vi "连续采集 - L1.vi"() -> ()   [LabVIEW 2017]
doc: "该范例演示了如何使用DAQmx设备进行连续带缓冲的电压测量。\n\n关于如何连接信号至DAQ设备，请查阅设备手册。"
uses:
  <vilib>/DAQmx/read.llb/DAQmx Read (Analog 2D DBL NChan NSamp).vi
  <vilib>/Analysis/baseanly.llb/Mean (DBL).vi
  <vilib>/DAQmx/write.llb/DAQmx Write (Digital U32 1Chan 1Samp).vi
  <vilib>/DAQmx/create/channels.llb/DAQmx Create Channel (DO-Digital Output).vi
  <vilib>/DAQmx/create/channels.llb/DAQmx Create Channel (AI-Voltage-Basic).vi
  <vilib>/DAQmx/configure/timing.llb/DAQmx Timing (Sample Clock).vi
  <vilib>/DAQmx/miscellaneous.llb/DAQmx Fill In Error Info.vi
  <resource>/objmgr/daqmx.rc
  <vilib>/Analysis/NI_AALBase.lvlib
  <vilib>/ptbypt/NI_PtbyPt.lvlib
panel:
  out "当前时间":timestamp
  out "实际间隔(s)":dbl=0.08 format="%.2g"
  out "显示队列中元素数量":i32
  in  "温度保存间隔(s)":dbl=0.08 format="%.2g"
  in  "校准间隔(s)":dbl=325.0
  out "mean":dbl caption="均值" format="%.7f"
  out "min value":dbl caption="最小值" format="%.7f"
  out "x-y":dbl
  out "校准进度":dbl(slide) scale=0.0..1.0 scale format="%%%#_6g"
  in  "信号采集设备":tag="Dev1"
  in  "波形查看":T1(tab)
  out "单环33":dbl
  out "单环22":dbl
  out "单环2":dbl[](graph)
  out "单环11":dbl
  out "单环3":dbl[](graph)
  out "单环1":dbl[](graph)
  out "单环55":dbl
  out "单环44":dbl
  out "单环5":dbl[](graph)
  out "单环4":dbl[](graph)
  out "N35":dbl=nan
  out "N34":dbl=nan
  out "N45":dbl=nan
  out "差分35":dbl[](graph)
  out "差分34":dbl[](graph)
  out "差分45":dbl[](graph)
  out "N25":dbl=nan
  out "N24":dbl=nan
  out "N23":dbl=nan
  out "差分25":dbl[](graph)
  out "差分24":dbl[](graph)
  out "差分23":dbl[](graph)
  out "N14":dbl=nan
  out "N13":dbl=nan
  out "N12":dbl=nan
  out "差分14":dbl[](graph)
  out "差分13":dbl[](graph)
  out "差分12":dbl[](graph)
  out "校准值":dbl[](array[numeric])
  out "N15":dbl=nan
  out "差分15":dbl[](graph)
  in  "开始":bool
  in  "波长":i32(ring)=3 items=["0"=-1, "1050"=0, "1213"=1, "1314"=2, "1409"=3, "1550"=4, "1609"=5]
  out "Order queue Name":string
  out "Inter queue Name":string
  out "系统标题":string
  out "序号":string
  in  "停止":bool
  # "RTC---"
  # "单环1"
  # "单环2"
  # "单环3"
  # "单环4"
  # "单环5"
  # "差分45"
  # "差分34"
  # "差分35"
  # "差分23"
  # "差分24"
  # "差分25"
  # "差分12"
  # "差分13"
  # "差分14"
  # "差分15"
  # "1环"
  # "2环"
  # "3环"
  # "4环"
  # "5环"
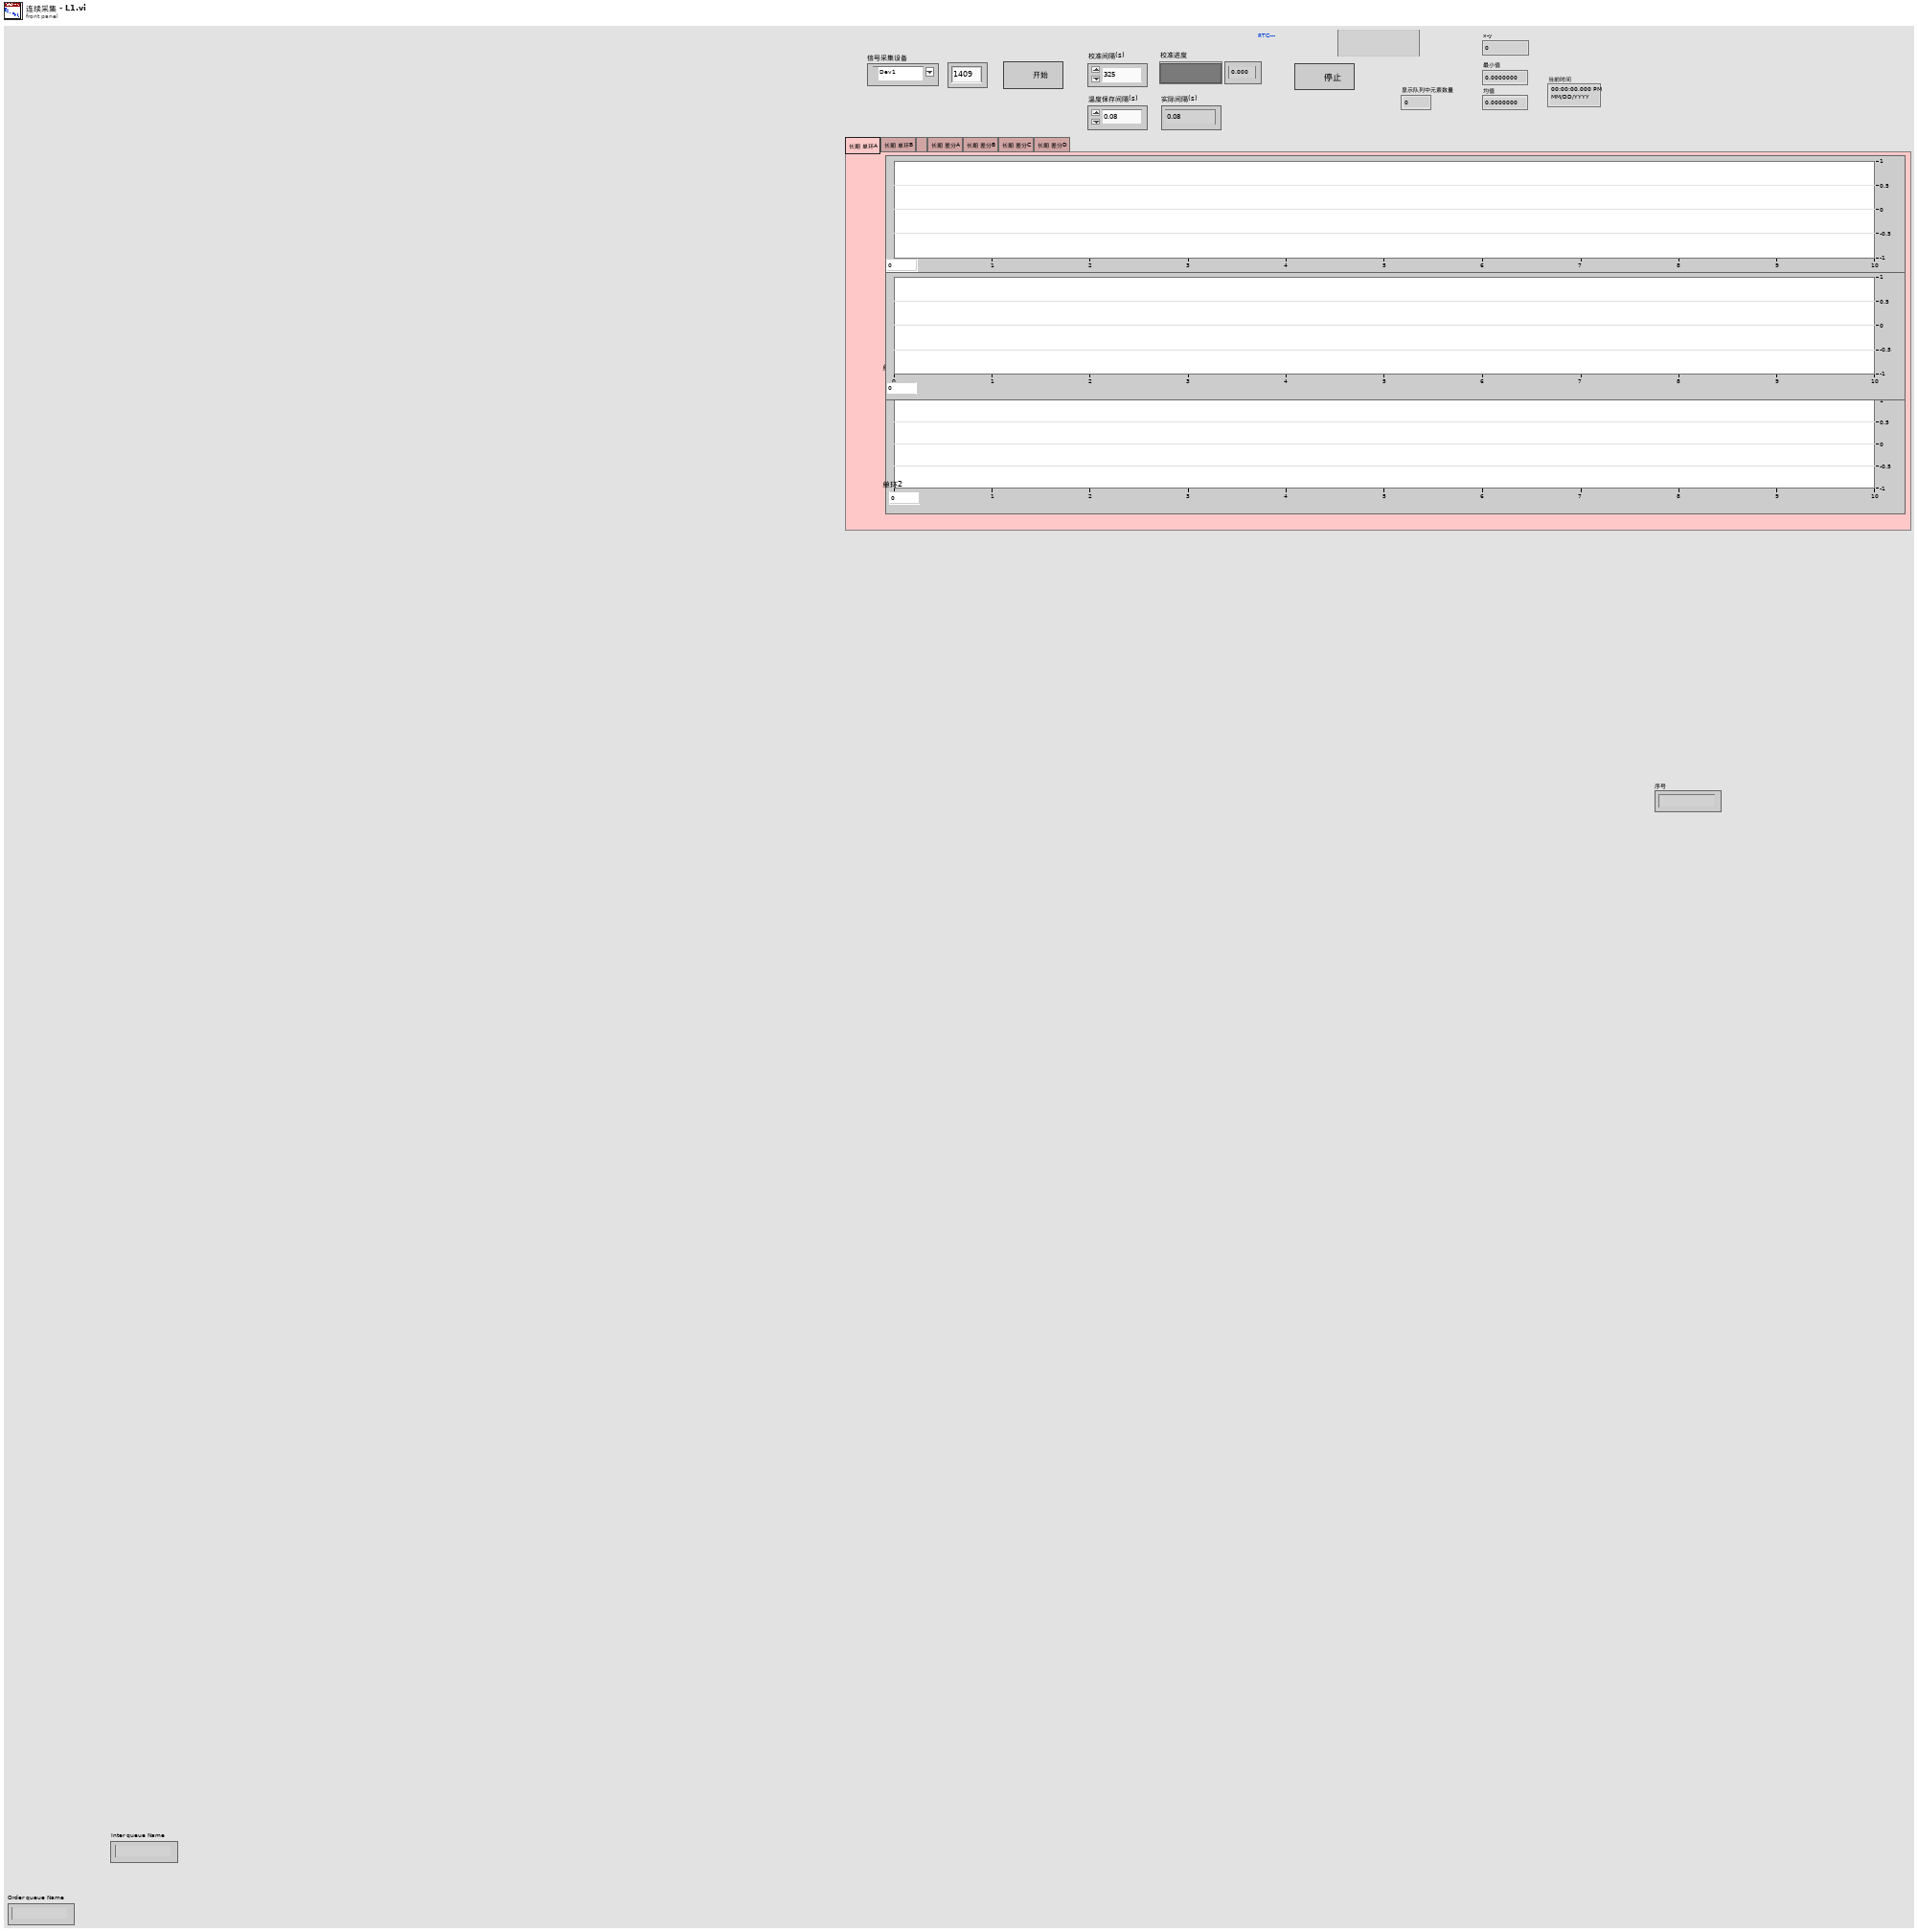
[diagram p1: front panel]
types:
  T1 = enum32{"长期 单环A", "长期 单环B", "  ", "长期 差分A", "长期 差分B", "长期 差分C", "长期 差分D"}
  T2 = cluster{"校准时间":timestamp, "tdms index":refnum<k34>, "Temp Title":string[], "温度保存间隔":dbl}
  T3 = typedef "用户事件自定义控件.ctl" = cluster{"消息":string, "指示":bool, "数据":dbl}
  T4 = cluster{"输入任务":refnum<k21>, "采样数":i32, "数字任务":refnum<k21>, "校准时间":timestamp, "校准值":dbl[], "数据路径":path}
  T5 = enum16{"open", "open or create", "create or replace", "create", "open (read-only)"}
  T6 = cluster{"温度采集":dbl[], "温度控制":dbl[], "压力测量":dbl[], "步进电机":dbl[], "湿度测量":dbl[], "LD温控":dbl[]}
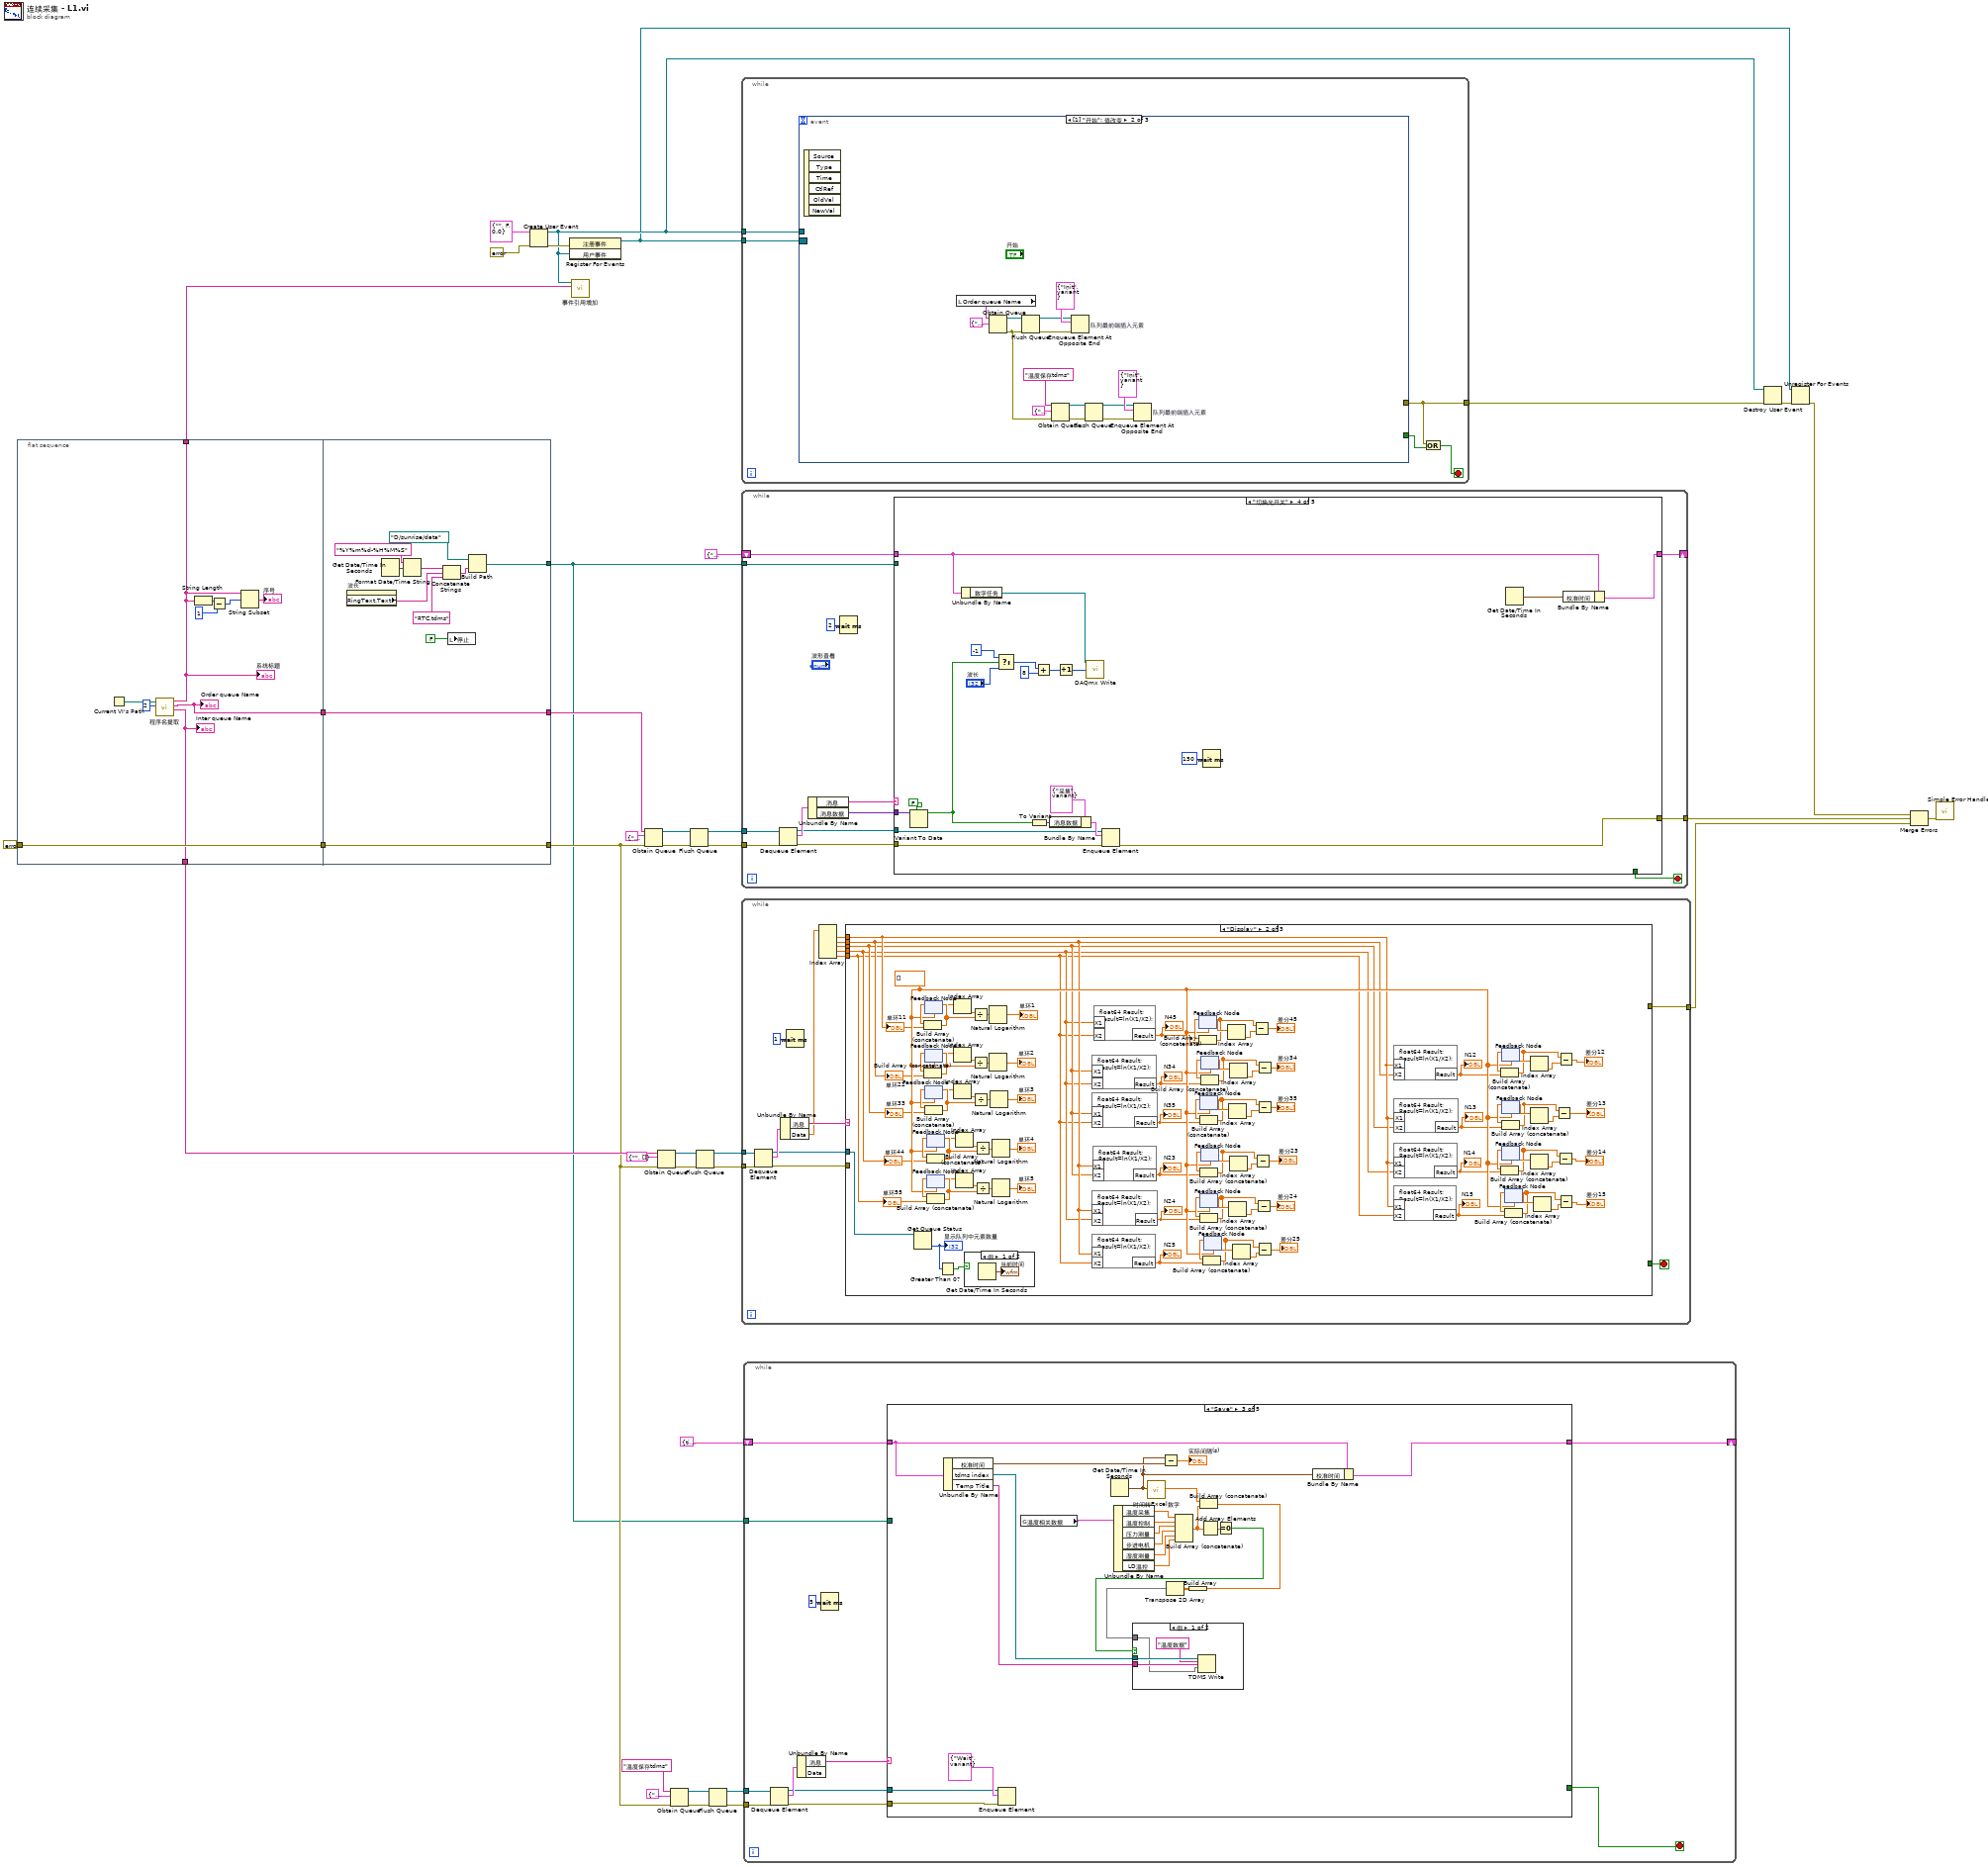
[diagram p0: block diagram]
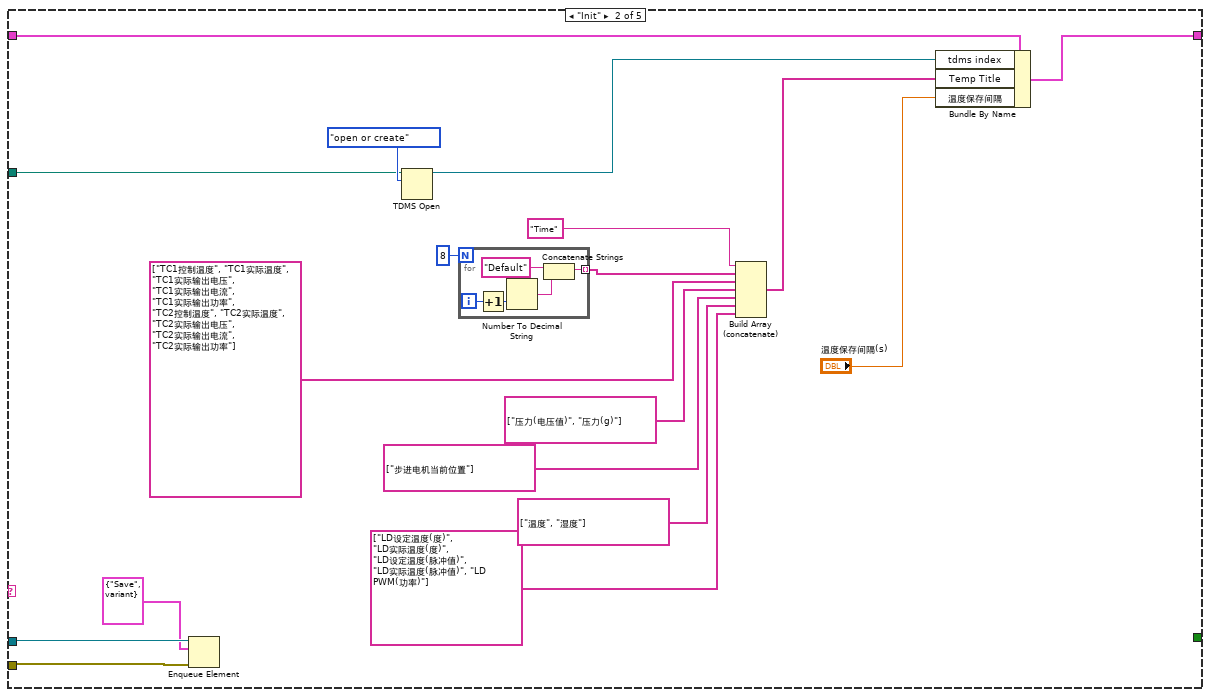
[diagram p3: hidden frame]
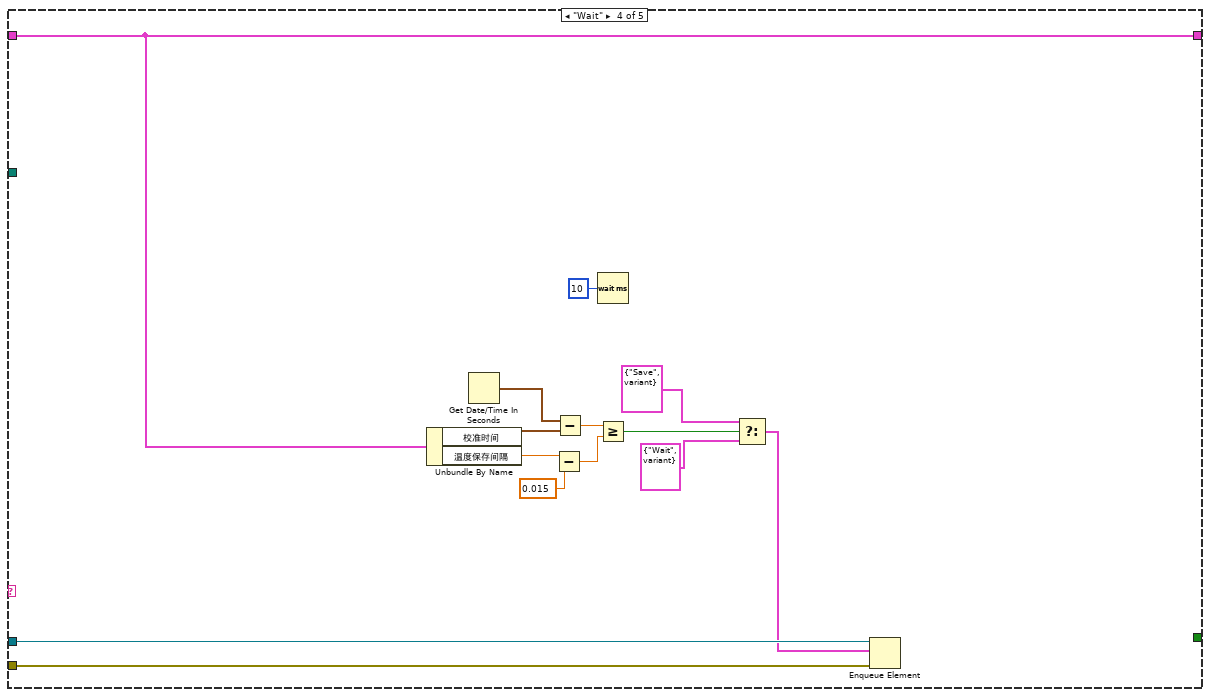
[diagram p5: hidden frame]
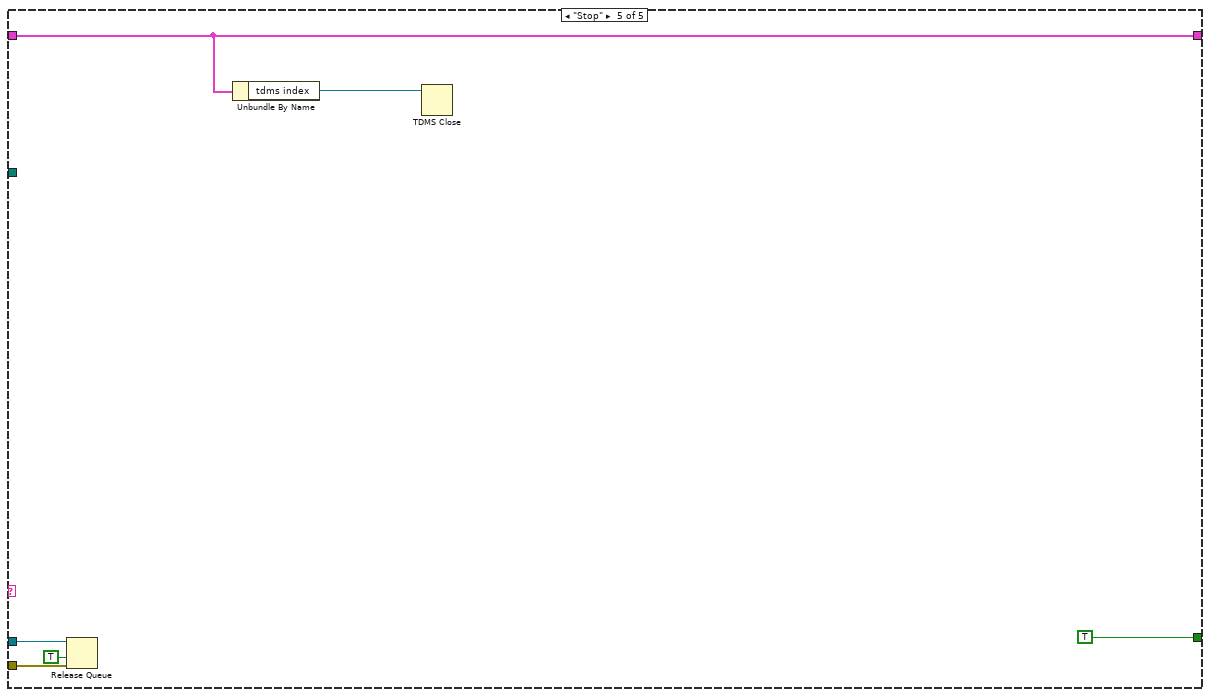
[diagram p6: hidden frame]
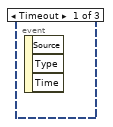
[diagram p7: hidden frame]
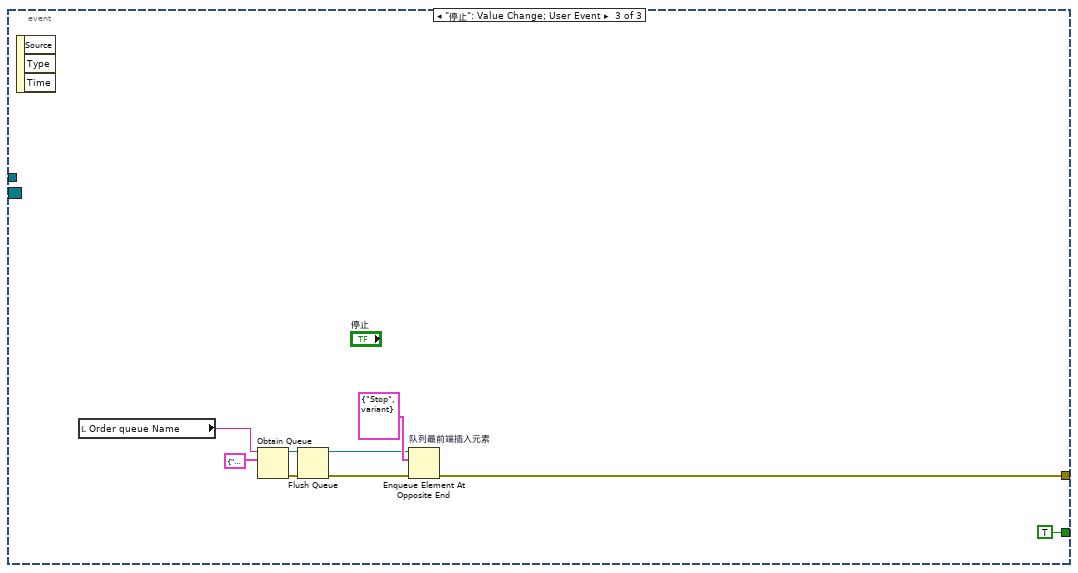
[diagram p8: hidden frame]
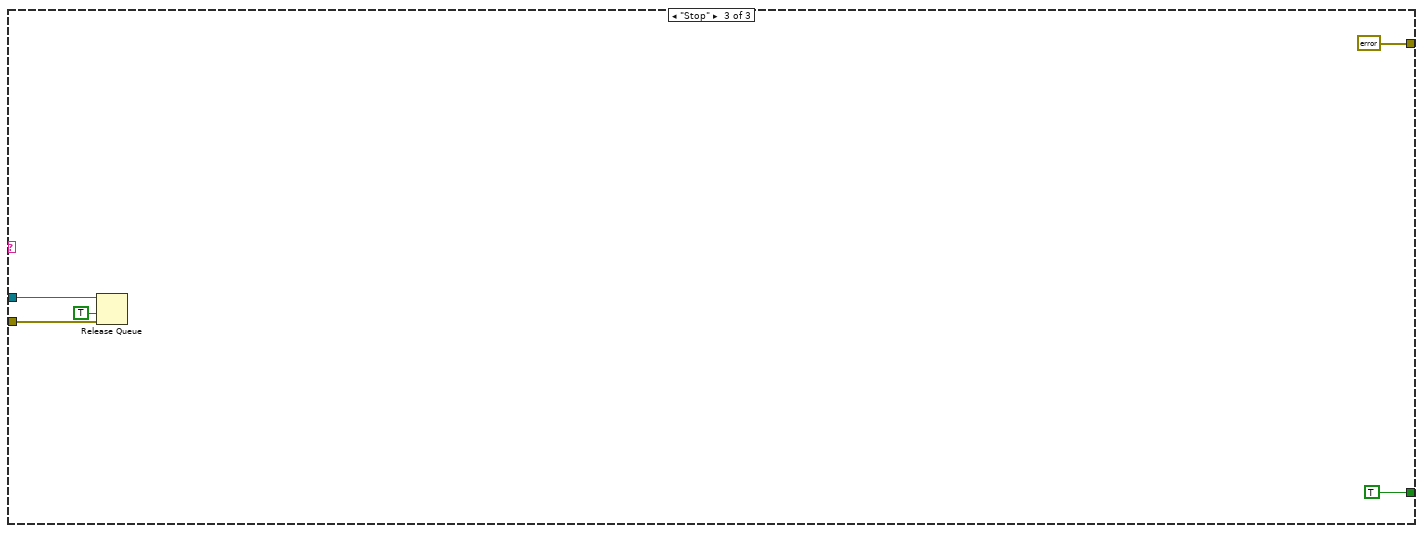
[diagram p11: hidden frame]
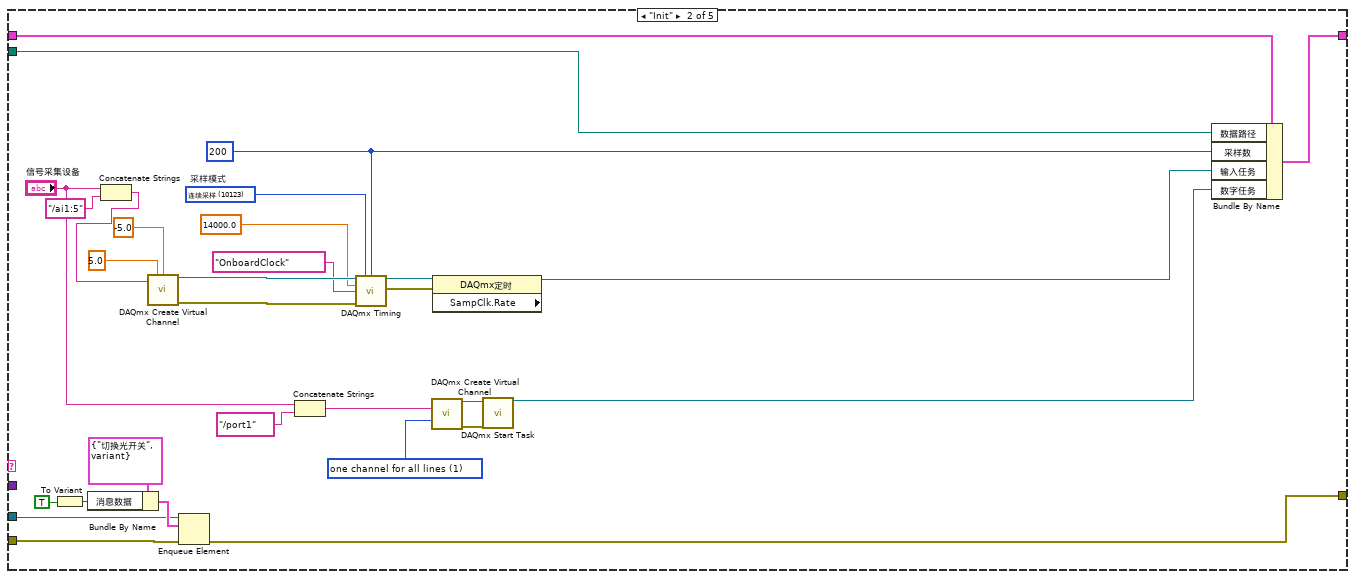
[diagram p13: hidden frame]
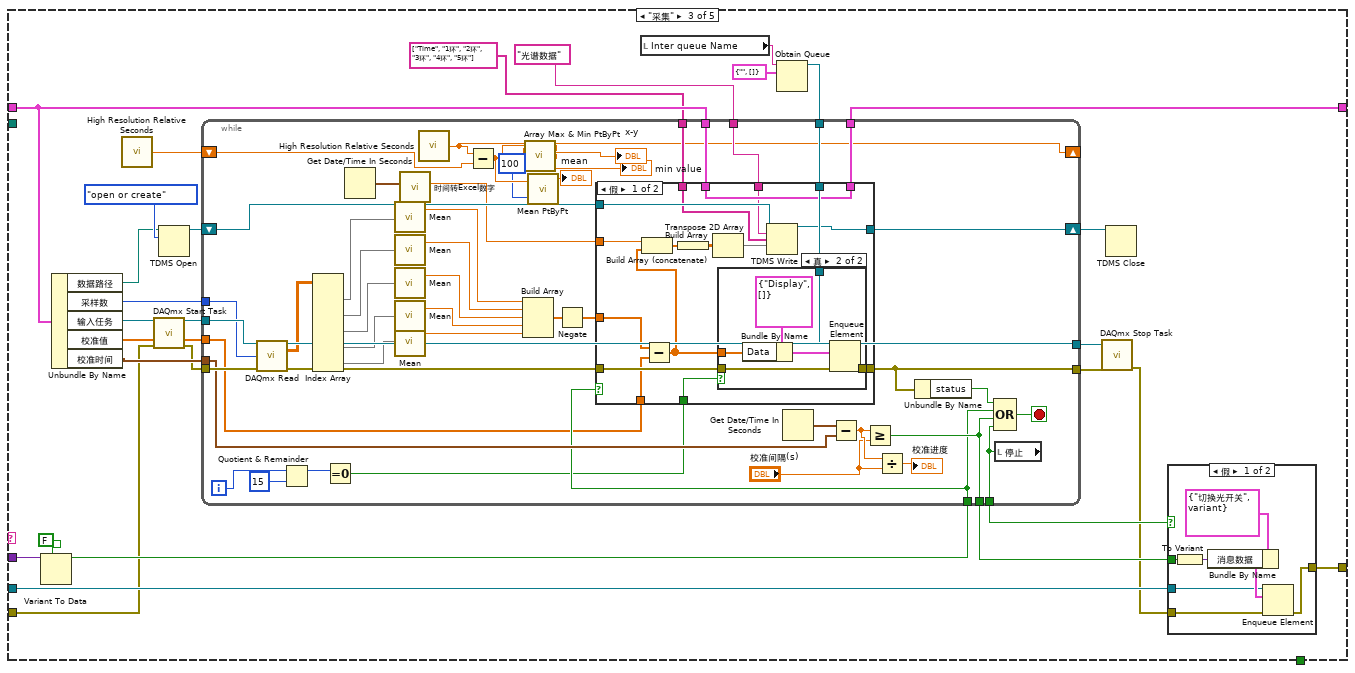
[diagram p14: hidden frame]
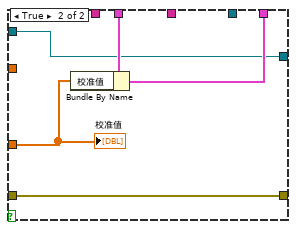
[diagram p17: hidden frame]
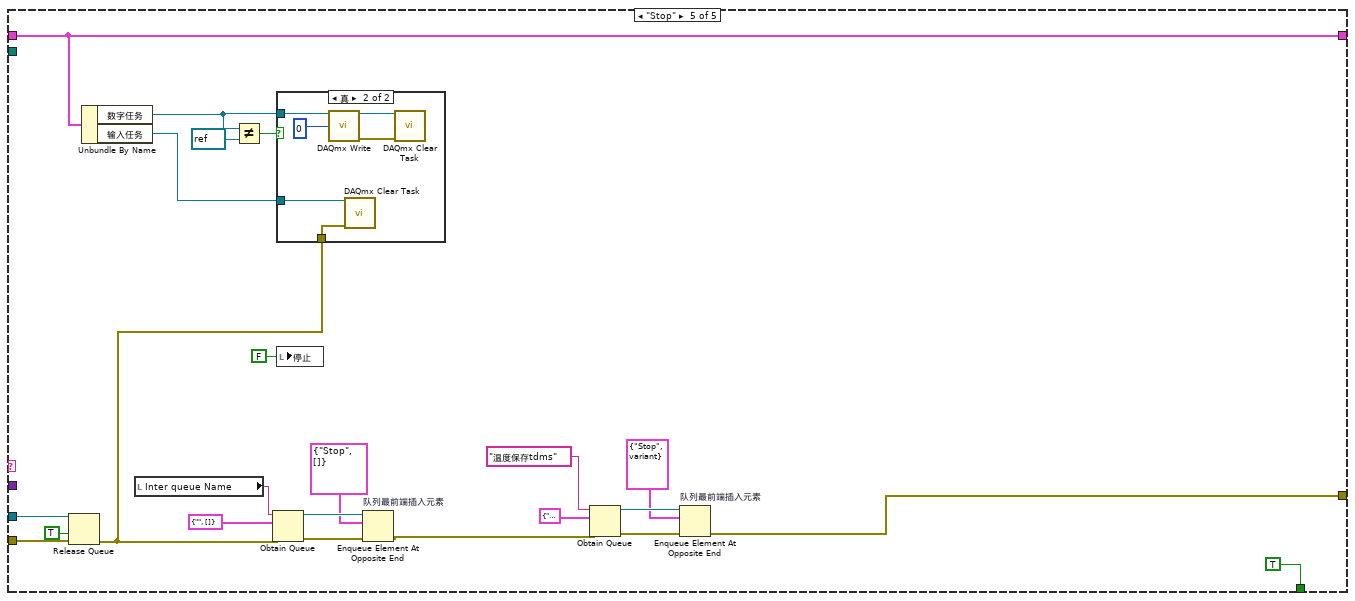
[diagram p18: hidden frame]
diagram:
  n1 = flat-sequence {
    tunnel: errorcluster {"status"=FALSE, "code"=0, "source"=""} ("错误常量") -> [w47]
    tunnel: [w47] -> w37
    tunnel: [w40] -> w24
    tunnel: [w39] -> w36
    tunnel: [w38] -> w16
    tunnel: [w58] -> w3
    tunnel: w37 -> [w58]
    tunnel: [w57] -> w31
    tunnel: w36 -> [w57]
    tunnel: [w50] -> w1
    frame #0 {
      n2 = Current VI's Path() -> (path=w46:path)
      n3 = call "程序名提取.vi"("标识长度"=2 ("长度"), "当前程序路径"=w46) -> ("Inter queue"=w38:string, "Order queue"=w39:string, "系统标题"=w40:string)  [unwired: 7 in]
      "Order queue Name" <- w39
      "Inter queue Name" <- w38
      "系统标题" <- w40
      n4 = String Length(string=w40) -> (length=w43:i32)
      n5 = Subtract(x=w43, y=1) -> (x-y=w44:i32)
      n6 = String Subset(string=w40, offset (0)=w44) -> (substring=→"序号":string)  [unwired: 1 in]
    }
    frame #1 {
      n7 = property on="波长" class="Ring (严格)"() -> ("RingText.Text"=w48:string)  [unwired: 2 in, 2 out]
      n8 = Get Date/Time In Seconds() -> (seconds since 1Jan1904=w52:timestamp)
      n9 = Format Date/Time String(time format string (%c)="%Y%m%d-%H%M%S" ("时间格式字符串(%c)"), seconds (now)=w52) -> (date/time string=w51:string)  [unwired: 1 in]
      n10 = Concatenate Strings(w51, w48, "RTC.tdms" ("字符串")) -> (w55:string)
      n11 = local write "停止"(FALSE ("暂停按钮")) -> ()
      n12 = Build Path(base path=path "D:/sunrise/data" ("存储路径"), name or relative path=w55) -> (appended path=w50:path)
    }
  }
  n13 = Create User Event(user event datatype=T3 {"消息"="", "指示"=FALSE, "数据"=0.0} ("用户事件"), error in=errorcluster {"status"=FALSE, "code"=0, "source"=""} ("错误输入（无错误）")) -> (user event=w22:refnum<user-event>, error out=w27:errorcluster)
  n14 = register-events(error in=w27, w22) -> (reference out=w21:refnum<event-registration>)  [unwired: 1 in, 1 out]
  n15 = call "事件引用增加.vi"("标识"=w24, "用户事件输入"=w22) -> ()  [unwired: 10 in]
  n16 = Obtain Queue(name (unnamed)=w31, element data type=cluster{"消息":string, "消息数据":variant} {"消息"="", "消息数据"=variant} ("Message Cluster"), error in (no error)=w3) -> (queue out=w33:refnum<queue>, error out=w32:errorcluster)  [unwired: 2 in, 1 out]
  n17 = Obtain Queue(name (unnamed)=w16, element data type=cluster{"消息":string, "Data":dbl[]} {"消息"="", "Data"=[]}, error in (no error)=w3) -> (queue out=w19:refnum<queue>, error out=w17:errorcluster)  [unwired: 2 in, 1 out]
  n18 = Obtain Queue(name (unnamed)="温度保存tdms" ("名称（未命名）"), element data type=cluster{"消息":string, "Data":variant} {"消息"="", "Data"=variant}, error in (no error)=w3) -> (queue out=w9:refnum<queue>, error out=w7:errorcluster)  [unwired: 2 in, 1 out]
  n19 = Flush Queue(queue=w33, error in (no error)=w32) -> (queue out=w30:refnum<queue>, error out=w29:errorcluster)  [unwired: 1 out]
  n20 = Flush Queue(queue=w19, error in (no error)=w17) -> (queue out=w12:refnum<queue>, error out=w11:errorcluster)  [unwired: 1 out]
  n21 = Flush Queue(queue=w9, error in (no error)=w7) -> (queue out=w6:refnum<queue>, error out=w5:errorcluster)  [unwired: 1 out]
  n22 = while {
    tunnel: w21 -> [w62]
    tunnel: w22 -> [w63]
    tunnel: [w59] -> w20
    stop <- w60 stop-if-true
    n23 = event shown="[1] \"开始\": 值改变" {
      selector: w62 -> [_ _ _]
      dyn-events: _ -> [_ _ _]
      timeout: _ -> [_ _ _]
      tunnel: w63 -> [_ _ _]
      tunnel: [_ _ w82] -> w59
      tunnel: [_ _ TRUE ("停止")] -> w61
      event Timeout {
        n24 = event-data() -> ()  [unwired: 1 in, 3 out]
      }
      event "开始": Value Change {
        n25 = event-data() -> ()  [unwired: 1 in, 6 out]
        n26 = local read "Order queue Name"() -> (w77:string)
        n27 = Obtain Queue(name (unnamed)=w77, element data type=cluster{"消息":string, "消息数据":variant} {"消息"="", "消息数据"=variant} ("Message Cluster")) -> (queue out=w74:refnum<queue>, error out=w65:errorcluster)  [unwired: 3 in, 1 out]
        n28 = Flush Queue(queue=w74, error in (no error)=w65) -> (queue out=w73:refnum<queue>, error out=w72:errorcluster)  [unwired: 1 out]
        n29 = Obtain Queue(name (unnamed)="温度保存tdms" ("名称（未命名）"), element data type=cluster{"消息":string, "消息数据":variant} {"消息"="", "消息数据"=variant} ("Message Cluster"), error in (no error)=w65) -> (queue out=w69:refnum<queue>, error out=w67:errorcluster)  [unwired: 2 in, 1 out]
        n30 = Enqueue Element At Opposite End "队列最前端插入元素"(queue=w73, element=cluster{"消息":string, "消息数据":variant} {"消息"="Init", "消息数据"=variant}, error in (no error)=w72) -> ()  [unwired: 1 in, 3 out]
        n31 = Flush Queue(queue=w69, error in (no error)=w67) -> (queue out=w68:refnum<queue>, error out=w66:errorcluster)  [unwired: 1 out]
        n32 = Enqueue Element At Opposite End "队列最前端插入元素"(queue=w68, element=cluster{"消息":string, "消息数据":variant} {"消息"="Init", "消息数据"=variant}, error in (no error)=w66) -> ()  [unwired: 1 in, 3 out]
      }
      event "停止": Value Change; User Event {
        n33 = event-data() -> ()  [unwired: 1 in, 3 out]
        n34 = local read "Order queue Name"() -> (w83:string)
        n35 = Obtain Queue(name (unnamed)=w83, element data type=cluster{"消息":string, "消息数据":variant} {"消息"="", "消息数据"=variant} ("Message Cluster")) -> (queue out=w84:refnum<queue>, error out=w79:errorcluster)  [unwired: 3 in, 1 out]
        n36 = Flush Queue(queue=w84, error in (no error)=w79) -> (queue out=w80:refnum<queue>, error out=w78:errorcluster)  [unwired: 1 out]
        n37 = Enqueue Element At Opposite End "队列最前端插入元素"(queue=w80, element=cluster{"消息":string, "消息数据":variant} {"消息"="Stop", "消息数据"=variant}, error in (no error)=w78) -> (error out=w82:errorcluster)  [unwired: 1 in, 2 out]
      }
    }
    n38 = Compound Arithmetic op=OR ("复合运算")(w59, w61) -> (w60:bool)
  }
  n39 = while {
    tunnel: w12 -> [w100]
    tunnel: w11 -> [w99]
    tunnel: [w88] -> w10
    stop <- w97 stop-if-true
    n40 = Dequeue Element(queue=w100, error in (no error)=w99) -> (queue out=w96:refnum<queue>, element=w101:cluster{"消息":string, "Data":dbl[]}, error out=w95:errorcluster)  [unwired: 1 in, 1 out]
    n41 = Unbundle By Name(w101) -> ("消息"=w98:string, "Data"=w94:dbl[])
    n42 = Wait (ms)(milliseconds to wait=u32 1 ("等待时间（毫秒）")) -> ()  [unwired: 1 out]
    n43 = Index Array(array=w94) -> (element #1=w93:dbl, element #2=w92:dbl, element #3=w91:dbl, element #4=w90:dbl, element #5=w89:dbl)  [unwired: 5 in]
    n44 = case shown="\"Display\"" w98 {
      tunnel: [_ _ TRUE] -> w97
      tunnel: w96 -> [_ w104 w189]
      tunnel: w95 -> [_ _ w188]
      tunnel: w93 -> [_ w120 _]
      tunnel: w92 -> [_ w119 _]
      tunnel: w91 -> [_ w118 _]
      tunnel: w90 -> [_ w117 _]
      tunnel: w89 -> [_ w116 _]
      tunnel: [_ _ errorcluster {"status"=FALSE, "code"=0, "source"=""} ("错误输入")] -> w88
      frame Default {
      }
      frame "Display" {
        w121 = dbl[] []
        n45 = Get Queue Status(queue=w104) -> (# elements in queue=w103:i32)  [unwired: 2 in, 7 out]
        "显示队列中元素数量" <- w103
        n46 = feedback #1(w121) -> (w182:dbl[])
        n47 = Build Array (concatenate)(w182, w120) -> (w183:dbl[])
        n48 = feedback-in #1(w183) -> ()
        n49 = feedback #2(w121) -> (w178:dbl[])
        n50 = Build Array (concatenate)(w178, w119) -> (w179:dbl[])
        n51 = feedback-in #2(w179) -> ()
        n52 = feedback #3(w121) -> (w173:dbl[])
        n53 = Build Array (concatenate)(w173, w118) -> (w174:dbl[])
        n54 = feedback-in #3(w174) -> ()
        n55 = feedback #4(w121) -> (w168:dbl[])
        n56 = Build Array (concatenate)(w168, w117) -> (w169:dbl[])
        n57 = feedback-in #4(w169) -> ()
        n58 = feedback #5(w121) -> (w163:dbl[])
        n59 = Build Array (concatenate)(w163, w116) -> (w164:dbl[])
        n60 = feedback-in #5(w164) -> ()
        n61 = Greater Than 0?(x=w103) -> (x > 0?=w102:bool)
        n62 = Index Array(array=w182) -> (element=w185:dbl)  [unwired: 1 in]
        n63 = Index Array(array=w178) -> (element=w181:dbl)  [unwired: 1 in]
        n64 = Index Array(array=w173) -> (element=w176:dbl)  [unwired: 1 in]
        n65 = Index Array(array=w168) -> (element=w171:dbl)  [unwired: 1 in]
        n66 = Index Array(array=w163) -> (element=w166:dbl)  [unwired: 1 in]
        n67 = case shown="假" w102 {
          frame False {
            n68 = Get Date/Time In Seconds() -> (seconds since 1Jan1904=→"当前时间":timestamp)
          }
          frame True {
          }
        }
        n69 = Divide(x=w185, y=w183) -> (x/y=w184:dbl[])
        n70 = Divide(x=w181, y=w179) -> (x/y=w180:dbl[])
        n71 = Divide(x=w176, y=w174) -> (x/y=w175:dbl[])
        n72 = Divide(x=w171, y=w169) -> (x/y=w170:dbl[])
        n73 = Divide(x=w166, y=w164) -> (x/y=w165:dbl[])
        n74 = Natural Logarithm(1:w184) -> (0:→"单环1":dbl[])
        n75 = Natural Logarithm(1:w180) -> (0:→"单环2":dbl[])
        n76 = Natural Logarithm(1:w175) -> (0:→"单环3":dbl[])
        n77 = Natural Logarithm(1:w170) -> (0:→"单环4":dbl[])
        n78 = Natural Logarithm(1:w165) -> (0:→"单环5":dbl[])
        n79 = formula code="float64 Result;\nResult=ln(X1/X2);"("X1"=w118, "X2"=w117) -> ("Result"=w114:dbl)
        "N34" <- w114
        n80 = formula code="float64 Result;\nResult=ln(X1/X2);"("X1"=w118, "X2"=w116) -> ("Result"=w113:dbl)
        "N35" <- w113
        n81 = formula code="float64 Result;\nResult=ln(X1/X2);"("X1"=w119, "X2"=w117) -> ("Result"=w111:dbl)
        "N24" <- w111
        n82 = formula code="float64 Result;\nResult=ln(X1/X2);"("X1"=w119, "X2"=w116) -> ("Result"=w110:dbl)
        "N25" <- w110
        n83 = formula code="float64 Result;\nResult=ln(X1/X2);"("X1"=w119, "X2"=w118) -> ("Result"=w112:dbl)
        "N23" <- w112
        n84 = formula code="float64 Result;\nResult=ln(X1/X2);"("X1"=w117, "X2"=w116) -> ("Result"=w115:dbl)
        "N45" <- w115
        n85 = feedback #6(w121) -> (w161:dbl[])
        n86 = Build Array (concatenate)(w161, w115) -> (w155:dbl[])
        n87 = feedback-in #6(w155) -> ()
        n88 = feedback #7(w121) -> (w159:dbl[])
        n89 = Build Array (concatenate)(w159, w113) -> (w148:dbl[])
        n90 = feedback-in #7(w148) -> ()
        n91 = feedback #8(w121) -> (w157:dbl[])
        n92 = Build Array (concatenate)(w157, w111) -> (w139:dbl[])
        n93 = feedback-in #8(w139) -> ()
        n94 = feedback #9(w121) -> (w158:dbl[])
        n95 = Build Array (concatenate)(w158, w112) -> (w144:dbl[])
        n96 = feedback-in #9(w144) -> ()
        n97 = feedback #10(w121) -> (w160:dbl[])
        n98 = Build Array (concatenate)(w160, w114) -> (w151:dbl[])
        n99 = feedback-in #10(w151) -> ()
        n100 = feedback #11(w121) -> (w156:dbl[])
        n101 = Build Array (concatenate)(w156, w110) -> (w141:dbl[])
        n102 = feedback-in #11(w141) -> ()
        n103 = Index Array(array=w161) -> (element=w154:dbl)  [unwired: 1 in]
        n104 = Index Array(array=w159) -> (element=w147:dbl)  [unwired: 1 in]
        n105 = Index Array(array=w157) -> (element=w138:dbl)  [unwired: 1 in]
        n106 = Index Array(array=w158) -> (element=w143:dbl)  [unwired: 1 in]
        n107 = Index Array(array=w160) -> (element=w150:dbl)  [unwired: 1 in]
        n108 = Index Array(array=w156) -> (element=w140:dbl)  [unwired: 1 in]
        n109 = Subtract(x=w155, y=w154) -> (x-y=→"差分45":dbl[])
        n110 = Subtract(x=w144, y=w143) -> (x-y=→"差分23":dbl[])
        n111 = Subtract(x=w139, y=w138) -> (x-y=→"差分24":dbl[])
        n112 = Subtract(x=w151, y=w150) -> (x-y=→"差分34":dbl[])
        n113 = Subtract(x=w148, y=w147) -> (x-y=→"差分35":dbl[])
        n114 = Subtract(x=w141, y=w140) -> (x-y=→"差分25":dbl[])
        n115 = formula code="float64 Result;\nResult=ln(X1/X2);"("X1"=w120, "X2"=w119) -> ("Result"=w109:dbl)
        "N12" <- w109
        n116 = formula code="float64 Result;\nResult=ln(X1/X2);"("X1"=w120, "X2"=w117) -> ("Result"=w107:dbl)
        "N14" <- w107
        n117 = formula code="float64 Result;\nResult=ln(X1/X2);"("X1"=w120, "X2"=w116) -> ("Result"=w106:dbl)
        "N15" <- w106
        n118 = formula code="float64 Result;\nResult=ln(X1/X2);"("X1"=w120, "X2"=w118) -> ("Result"=w108:dbl)
        "N13" <- w108
        n119 = feedback #12(w121) -> (w137:dbl[])
        n120 = Build Array (concatenate)(w137, w109) -> (w133:dbl[])
        n121 = feedback-in #12(w133) -> ()
        n122 = feedback #13(w121) -> (w135:dbl[])
        n123 = Build Array (concatenate)(w135, w107) -> (w127:dbl[])
        n124 = feedback-in #13(w127) -> ()
        n125 = feedback #14(w121) -> (w136:dbl[])
        n126 = Build Array (concatenate)(w136, w108) -> (w131:dbl[])
        n127 = feedback-in #14(w131) -> ()
        n128 = feedback #15(w121) -> (w134:dbl[])
        n129 = Build Array (concatenate)(w134, w106) -> (w129:dbl[])
        n130 = feedback-in #15(w129) -> ()
        n131 = Index Array(array=w137) -> (element=w132:dbl)  [unwired: 1 in]
        n132 = Index Array(array=w135) -> (element=w126:dbl)  [unwired: 1 in]
        n133 = Index Array(array=w136) -> (element=w130:dbl)  [unwired: 1 in]
        n134 = Index Array(array=w134) -> (element=w128:dbl)  [unwired: 1 in]
        n135 = Subtract(x=w131, y=w130) -> (x-y=→"差分13":dbl[])
        n136 = Subtract(x=w127, y=w126) -> (x-y=→"差分14":dbl[])
        n137 = Subtract(x=w133, y=w132) -> (x-y=→"差分12":dbl[])
        n138 = Subtract(x=w129, y=w128) -> (x-y=→"差分15":dbl[])
        "单环11" <- w120
        "单环22" <- w119
        "单环33" <- w118
        "单环44" <- w117
        "单环55" <- w116
      }
      frame "Stop" {
        n139 = Release Queue(queue=w189, force destroy? (F)=TRUE ("强制销毁？(F)"), error in (no error)=w188) -> ()  [unwired: 3 out]
      }
    }
  }
  n140 = while {
    tunnel: w30 -> [w204]
    tunnel: w29 -> [w203]
    shift-right: [w199] -> _
    shift-left: T4 {"输入任务"="", "采样数"=100, "数字任务"="", "校准时间"=timestamp(0 s since 1904-01-01), "校准值"=[0.0, 0.0, 0.0, 0.0, 0.0], "数据路径"=path ""} -> [w200]
    tunnel: [w195] -> w13
    tunnel: w1 -> [w192]
    stop <- w196 stop-if-true
    n141 = Dequeue Element(queue=w204, error in (no error)=w203) -> (queue out=w198:refnum<queue>, element=w202:cluster{"消息":string, "消息数据":variant}, error out=w197:errorcluster)  [unwired: 1 in, 1 out]
    n142 = Unbundle By Name(w202) -> ("消息"=w201:string, "消息数据"=w194:variant)
    n143 = Wait (ms)(milliseconds to wait=u32 2 ("等待时间（毫秒）")) -> ()  [unwired: 1 out]
    n144 = case shown="\"切换光开关\"" w201 {
      tunnel: w200 -> [w206 w225 w252 w362 w388]
      tunnel: [w206 w223 w251 w360 w388] -> w199
      tunnel: w198 -> [_ w210 w261 w356 w390]
      tunnel: w197 -> [w205 w212 w248 w355 w389]
      tunnel: [_ _ _ _ TRUE] -> w196
      tunnel: [w205 w211 w260 w354 w374] -> w195
      tunnel: w194 -> [_ _ w264 w364 _]
      tunnel: w192 -> [_ w207 _ _ _]
      frame Default {
      }
      frame "Init" {
        w220 = 1 items=["one channel for each line", "one channel for all lines"] ("line grouping")
        w224 = 200 ("采样数")
        w234 = 10123 items=["有限采样"=10178, "连续采样"=10123, "硬件定时单点"=12522]  # 采样模式
        n145 = To Variant(anything=TRUE) -> (Variant=w215:variant)
        n146 = Bundle By Name(cluster=cluster{"消息":string, "消息数据":variant} {"消息"="切换光开关", "消息数据"=variant} ("element"), "消息数据"=w215) -> (w216:cluster{"消息":string, "消息数据":variant})
        n147 = Concatenate Strings("信号采集设备", "/ai1:5" ("字符串")) -> (w226:string)
        n148 = call-poly <vilib>:"DAQmx Create Virtual Channel.vi"("maximum value"=5.0 ("最大电压"), "minimum value"=-5.0 ("最小电压"), "physical channels"=w226) -> ("task out"=w232:refnum<k21>, "error out"=w233:errorcluster)  [unwired: 11 in]
        n149 = Enqueue Element(queue=w210, element=w216, error in (no error)=w212) -> (error out=w211:errorcluster)  [unwired: 1 in, 2 out]
        n150 = Concatenate Strings("信号采集设备", "/port1" ("字符串")) -> (w218:string)
        n151 = call-poly <vilib>:"DAQmx Timing.vi"("task/channels in"=w232, "sample mode"=w234, "samples per channel"=w224, "rate"=14000.0 ("采样率"), "source"=tag "OnboardClock" ("采样时钟源"), "error in"=w233) -> ("task out"=w236:refnum<k21>, "error out"=w235:errorcluster)  [unwired: 8 in]
        n152 = call-poly <vilib>:"DAQmx Create Virtual Channel.vi"("lines"=w218, "line grouping"=w220) -> ("task out"=w221:refnum<k21>, "error out"=w222:errorcluster)  [unwired: 12 in]
        n153 = property class="DAQmx定时" props=["SampClk.Rate"](reference=w236, error in=w235) -> (reference out=w208:refnum<k21>)  [unwired: 2 out]
        n154 = call <vilib>:"DAQmx Start Task.vi"("task/channels in"=w221, "error in"=w222) -> ("task out"=w217:refnum<k21>)  [unwired: 12 in, 1 out]
        n155 = Bundle By Name(cluster=w225, "数据路径"=w207, "采样数"=w224, "输入任务"=w208, "数字任务"=w217) -> (w223:T4)
      }
      frame "采集" {
        n156 = Variant To Data(type=FALSE, Variant=w264) -> (data=w262:bool)  [unwired: 1 in, 1 out]
        n157 = Unbundle By Name(w252) -> ("数据路径"=w242:path, "采样数"=w265:i32, "输入任务"=w250:refnum<k21>, "校准值"=w253:dbl[], "校准时间"=w254:timestamp)
        n158 = call <vilib>:"High Resolution Relative Seconds.vi"() -> ("relative seconds"=w237:dbl)
        n159 = call <vilib>:"DAQmx Start Task.vi"("task/channels in"=w250, "error in"=w248) -> ("task out"=w249:refnum<k21>, "error out"=w247:errorcluster)  [unwired: 12 in]
        n160 = TDMS Open(10:T5."open or create" ("操作(0:open)"), 11:w242) -> (3:w240:refnum<k34>)  [unwired: 5 in, 1 out]
        n161 = local read "Inter queue Name"() -> (w257:string)
        n162 = Obtain Queue(name (unnamed)=w257, element data type=cluster{"消息":string, "Data":dbl[]} {"消息"="", "Data"=[]}) -> (queue out=w255:refnum<queue>)  [unwired: 3 in, 2 out]
        n163 = while {
          tunnel: w249 -> [w323]
          tunnel: [w322] -> w246
          tunnel: [w311] -> w245
          tunnel: w265 -> [w319]
          tunnel: w247 -> [w318]
          tunnel: w262 -> [w306]
          tunnel: [w315] -> w259
          tunnel: w254 -> [w316]
          tunnel: [w314] -> w258
          tunnel: w255 -> [w313]
          tunnel: w253 -> [w278]
          tunnel: w252 -> [w308]
          tunnel: [w307] -> w251
          shift-right: [w302] -> w241
          shift-left: w240 -> [w301]
          tunnel: "光谱数据" ("组名称输入（无标题）") -> [w300]
          tunnel: string[] ["Time", "1环", "2环", "3环", "4环", "5环"] ("通道名输入（无标题）") -> [w299]
          shift-right: [w285] -> _
          shift-left: w237 -> [w286]
          i -> [w277]
          stop <- w320 stop-if-true
          w281 = 100 ("sample length")
          n164 = call-poly <vilib>:"DAQmx Read.vi"("task/channels in"=w323, "number of samples per channel"=w319, "error in"=w318) -> ("task out"=w322:refnum<k21>, "data"=w310:dbl[][], "error out"=w312:errorcluster)  [unwired: 10 in]
          n165 = Quotient & Remainder(x=w277, y=15) -> (x-y*floor(x/y)=w275:i32)  [unwired: 1 out]
          n166 = Index Array(array=w310) -> (element #1=w293:dbl[], element #2=w292:dbl[], element #3=w291:dbl[], element #4=w290:dbl[], element #5=w289:dbl[])  [unwired: 10 in]
          n167 = Equal To 0?(x=w275) -> (x = 0?=w274:bool)
          n168 = Get Date/Time In Seconds() -> (seconds since 1Jan1904=w288:timestamp)
          n169 = call-poly <vilib>:"Mean.vi"("X"=w293) -> ("mean"=w298:dbl)  [unwired: 1 out]
          n170 = call-poly <vilib>:"Mean.vi"("X"=w292) -> ("mean"=w297:dbl)  [unwired: 1 out]
          n171 = call-poly <vilib>:"Mean.vi"("X"=w291) -> ("mean"=w296:dbl)  [unwired: 1 out]
          n172 = call-poly <vilib>:"Mean.vi"("X"=w290) -> ("mean"=w295:dbl)  [unwired: 1 out]
          n173 = call-poly <vilib>:"Mean.vi"("X"=w289) -> ("mean"=w294:dbl)  [unwired: 1 out]
          n174 = call "时间转Excel数字.vi"("温湿度采集时刻"=w288) -> ("数值"=w287:dbl)  [unwired: 10 in]
          n175 = call <vilib>:"High Resolution Relative Seconds.vi"() -> ("relative seconds"=w285:dbl)
          n176 = Subtract(x=w285, y=w286) -> (x-y=w282:dbl)
          n177 = Build Array(w298, w297, w296, w295, w294) -> (w309:dbl[])
          n178 = call <vilib>:"Array Max & Min PtByPt.vi"("input data point"=w282, "sample length"=w281) -> ("max value"=→"x-y":dbl, "min value"=→"min value":dbl)  [unwired: 1 in, 3 out]
          n179 = call <vilib>:"Mean PtByPt.vi"("x"=w282, "sample length"=w281) -> ("mean"=→"mean":dbl)  [unwired: 2 in, 1 out]
          n180 = Negate(x=w309) -> (-x=w305:dbl[])
          n181 = case shown="假" w306 {
            tunnel: w313 -> [w339 _]
            tunnel: w312 -> [w338 w349]
            tunnel: [w337 w349] -> w311
            tunnel: w278 -> [w336 _]
            tunnel: w301 -> [w335 w347]
            tunnel: w305 -> [w334 w348]
            tunnel: w308 -> [w333 w351]
            tunnel: [w333 w350] -> w307
            tunnel: [w332 w347] -> w302
            tunnel: w300 -> [w331 _]
            tunnel: w299 -> [w330 _]
            tunnel: w287 -> [w327 _]
            tunnel: w274 -> [w324 _]
            frame False {
              n182 = Subtract(x=w334, y=w336) -> (x-y=w326:dbl[])
              n183 = Build Array (concatenate)(w327, w326) -> (w329:dbl[])
              n184 = Build Array(w329) -> (w328:dbl[][])
              n185 = Transpose 2D Array(2D array=w328) -> (transposed array=w325:dbl[][])
              n186 = case shown="真" w324 {
                tunnel: w339 -> [_ w346]
                tunnel: w338 -> [w340 w345]
                tunnel: [w340 w344] -> w337
                tunnel: w326 -> [_ w341]
                frame False {
                }
                frame True {
                  n187 = Bundle By Name(cluster=cluster{"消息":string, "Data":dbl[]} {"消息"="Display", "Data"=[]}, "Data"=w341) -> (w342:cluster{"消息":string, "Data":dbl[]})
                  n188 = Enqueue Element(queue=w346, element=w342, error in (no error)=w345) -> (error out=w344:errorcluster)  [unwired: 1 in, 2 out]
                }
              }
              n189 = TDMS Write(0:w335, 5:w331, 7:w330, 9:w325) -> (4:w332:refnum<k34>)  [unwired: 2 in, 3 out]
            }
            frame True {
              n190 = Bundle By Name(cluster=w351, "校准值"=w348) -> (w350:T4)
              "校准值" <- w348
            }
          }
          n191 = Get Date/Time In Seconds() -> (seconds since 1Jan1904=w317:timestamp)
          n192 = Subtract(x=w317, y=w316) -> (x-y=w304:dbl)
          n193 = Greater Or Equal?(x=w304, y="校准间隔(s)") -> (x >= y?=w314:bool)
          n194 = Divide(x=w304, y="校准间隔(s)") -> (x/y=→"校准进度":dbl)
          n195 = Unbundle By Name(w311) -> ("status"=w321:bool)
          n196 = local read "停止"() -> (w315:bool)
          n197 = Compound Arithmetic op=OR ("复合运算")(w321, w306, w314, w315) -> (w320:bool)
        }
        n198 = call <vilib>:"DAQmx Stop Task.vi"("task/channels in"=w246, "error in"=w245) -> ("error out"=w244:errorcluster)  [unwired: 12 in, 1 out]
        n199 = TDMS Close(11:w241) -> ()  [unwired: 1 in, 2 out]
        n200 = case shown="假" w259 {
          tunnel: w261 -> [w269 _]
          tunnel: w244 -> [w268 w273]
          tunnel: [w267 w273] -> w260
          tunnel: w258 -> [w266 _]
          frame False {
            n201 = To Variant(anything=w266) -> (Variant=w271:variant)
            n202 = Bundle By Name(cluster=cluster{"消息":string, "消息数据":variant} {"消息"="切换光开关", "消息数据"=variant} ("element"), "消息数据"=w271) -> (w272:cluster{"消息":string, "消息数据":variant})
            n203 = Enqueue Element(queue=w269, element=w272, error in (no error)=w268) -> (error out=w267:errorcluster)  [unwired: 1 in, 2 out]
          }
          frame True {
          }
        }
      }
      frame "切换光开关" {
        n204 = Variant To Data(type=FALSE, Variant=w364) -> (data=w353:bool)  [unwired: 1 in, 1 out]
        n205 = Unbundle By Name(w362) -> ("数字任务"=w363:refnum<k21>)
        n206 = Select(t=-1 ("f"), s=w353, f="波长") -> (s? t:f=w367:i32)
        n207 = To Variant(anything=w353) -> (Variant=w358:variant)
        n208 = Add(x=w367, y=8) -> (x+y=w370:i32)
        n209 = Bundle By Name(cluster=cluster{"消息":string, "消息数据":variant} {"消息"="采集", "消息数据"=variant} ("element"), "消息数据"=w358) -> (w359:cluster{"消息":string, "消息数据":variant})
        n210 = Increment(x=w370) -> (x+1=w371:i32)
        n211 = call-poly <vilib>:"DAQmx Write.vi"("task/channels in"=w363, "data"=w371) -> ()  [unwired: 11 in, 3 out]
        n212 = Enqueue Element(queue=w356, element=w359, error in (no error)=w355) -> (error out=w354:errorcluster)  [unwired: 1 in, 2 out]
        n213 = Wait (ms)(milliseconds to wait=u32 150 ("等待时间（毫秒）")) -> ()  [unwired: 1 out]
        n214 = Get Date/Time In Seconds() -> (seconds since 1Jan1904=w361:timestamp)
        n215 = Bundle By Name(cluster=w362, "校准时间"=w361) -> (w360:T4)
      }
      frame "Stop" {
        n216 = Release Queue(queue=w390, force destroy? (F)=TRUE ("强制销毁？(F)"), error in (no error)=w389) -> (error out=w379:errorcluster)  [unwired: 2 out]
        n217 = Unbundle By Name(w388) -> ("数字任务"=w386:refnum<k21>, "输入任务"=w380:refnum<k21>)
        n218 = local read "Inter queue Name"() -> (w381:string)
        n219 = Not Equal?(x=w386, y=refnum<k21> refnum ("数字任务")) -> (x != y?=w385:bool)
        n220 = Obtain Queue(name (unnamed)=w381, element data type=cluster{"消息":string, "Data":dbl[]} {"消息"="", "Data"=[]}, error in (no error)=w379) -> (queue out=w394:refnum<queue>, error out=w393:errorcluster)  [unwired: 2 in, 1 out]
        n221 = case shown="真" w385 {
          tunnel: w386 -> [_ w397]
          tunnel: w380 -> [_ w396]
          tunnel: w379 -> [_ w395]
          frame False {
          }
          frame True {
            n222 = call-poly <vilib>:"DAQmx Write.vi"("task/channels in"=w397, "data"=u32 0) -> ("task out"=w400:refnum<k21>, "error out"=w399:errorcluster)  [unwired: 11 in, 1 out]
            n223 = call <vilib>:"DAQmx Clear Task.vi"("task in"=w396, "error in"=w395) -> ()  [unwired: 13 in, 1 out]
            n224 = call <vilib>:"DAQmx Clear Task.vi"("task in"=w400, "error in"=w399) -> ()  [unwired: 13 in, 1 out]
          }
        }
        n225 = local write "停止"(FALSE) -> ()
        n226 = Enqueue Element At Opposite End "队列最前端插入元素"(queue=w394, element=cluster{"消息":string, "Data":dbl[]} {"消息"="Stop", "Data"=[]}, error in (no error)=w393) -> (error out=w376:errorcluster)  [unwired: 1 in, 2 out]
        n227 = Obtain Queue(name (unnamed)="温度保存tdms" ("名称（未命名）"), element data type=cluster{"消息":string, "Data":variant} {"消息"="", "Data"=variant}, error in (no error)=w376) -> (queue out=w377:refnum<queue>, error out=w378:errorcluster)  [unwired: 2 in, 1 out]
        n228 = Enqueue Element At Opposite End "队列最前端插入元素"(queue=w377, element=cluster{"消息":string, "Data":variant} {"消息"="Stop", "Data"=variant}, error in (no error)=w378) -> (error out=w374:errorcluster)  [unwired: 1 in, 2 out]
      }
    }
  }
  n229 = while {
    tunnel: w6 -> [w410]
    tunnel: w5 -> [w409]
    shift-right: [w404] -> _
    shift-left: T2 {"校准时间"=timestamp(0 s since 1904-01-01), "tdms index"=refnum, "Temp Title"=[], "温度保存间隔"=0.1} -> [w405]
    tunnel: w1 -> [w401]
    stop <- w403 stop-if-true
    n230 = Dequeue Element(queue=w410, error in (no error)=w409) -> (queue out=w407:refnum<queue>, element=w411:cluster{"消息":string, "Data":variant}, error out=w406:errorcluster)  [unwired: 1 in, 1 out]
    n231 = Unbundle By Name(w411) -> ("消息"=w408:string)  [unwired: 1 out]
    n232 = Wait (ms)(milliseconds to wait=u32 5 ("等待时间（毫秒）")) -> ()  [unwired: 1 out]
    n233 = case shown="\"Save\"" w408 {
      tunnel: w407 -> [_ w429 w442 w467 w482]
      tunnel: w406 -> [_ w428 w441 w466 w481]
      tunnel: w405 -> [w412 w426 w459 w469 w479]
      tunnel: [w412 w424 w458 w469 w479] -> w404
      tunnel: [_ _ _ _ TRUE] -> w403
      tunnel: w401 -> [_ w414 _ _ _]
      frame Default {
      }
      frame "Init" {
        n234 = Enqueue Element(queue=w429, element=cluster{"消息":string, "消息数据":variant} {"消息"="Save", "消息数据"=variant}, error in (no error)=w428) -> ()  [unwired: 1 in, 3 out]
        n235 = TDMS Open(10:T5."open or create" ("操作(0:open)"), 11:w414) -> (3:w425:refnum<k34>)  [unwired: 5 in, 1 out]
        n236 = for {
          N: 8 -> [_]
          tunnel: [w431] -> w416 mode=indexing
          i -> [w435]
          n237 = Increment(x=w435) -> (x+1=w434:i32)
          n238 = Number To Decimal String(number=w434) -> (decimal integer string=w433:string)  [unwired: 1 in]
          n239 = Concatenate Strings("Default", w433) -> (w431:string)
        }
        n240 = Build Array (concatenate)("Time", w416, string[] ["TC1控制温度", "TC1实际温度", "TC1实际输出电压", "TC1实际输出电流", "TC1实际输出功率", "TC2控制温度", "TC2实际温度", "TC2实际输出电压", "TC2实际输出电流", "TC2实际输出功率"], string[] ["压力(电压值)", "压力(g)"], string[] ["步进电机当前位置"], string[] ["温度", "湿度"], string[] ["LD设定温度(度)", "LD实际温度(度)", "LD设定温度(脉冲值)", "LD实际温度(脉冲值)", "LD PWM(功率)"]) -> (w418:string[])
        n241 = Bundle By Name(cluster=w426, "tdms index"=w425, "Temp Title"=w418, "温度保存间隔"="温度保存间隔(s)") -> (w424:T2)
      }
      frame "Save" {
        n242 = Unbundle By Name(w459) -> ("校准时间"=w438:timestamp, "tdms index"=w457:refnum<k34>, "Temp Title"=w456:string[])
        n243 = Enqueue Element(queue=w442, element=cluster{"消息":string, "消息数据":variant} {"消息"="Wait", "消息数据"=variant}, error in (no error)=w441) -> ()  [unwired: 1 in, 3 out]
        n244 = global read "辅助系统全局变量 - T2.vi" "温度相关数据"() -> (w444:T6)
        n245 = Get Date/Time In Seconds() -> (seconds since 1Jan1904=w437:timestamp)
        n246 = Unbundle By Name(w444) -> ("温度采集"=w455:dbl[], "温度控制"=w454:dbl[], "压力测量"=w453:dbl[], "步进电机"=w452:dbl[], "湿度测量"=w451:dbl[], "LD温控"=w450:dbl[])
        n247 = call "时间转Excel数字.vi"("温湿度采集时刻"=w437) -> ("数值"=w448:dbl)  [unwired: 10 in]
        n248 = Subtract(x=w437, y=w438) -> (x-y=→"实际间隔(s)":dbl)
        n249 = Build Array (concatenate)(w455, w454, w453, w452, w451, w450) -> (w447:dbl[])
        n250 = Build Array (concatenate)(w448, w447) -> (w445:dbl[])
        n251 = Build Array(w445) -> (w440:dbl[][])
        n252 = Transpose 2D Array(2D array=w440) -> (transposed array=w439:dbl[][])
        n253 = Add Array Elements(numeric array=w447) -> (sum=w449:dbl)
        n254 = Equal To 0?(x=w449) -> (x = 0?=w446:bool)
        n255 = case shown="假" w446 {
          tunnel: w457 -> [w463 _]
          tunnel: w456 -> [w462 _]
          tunnel: w439 -> [w460 _]
          frame False {
            n256 = TDMS Write(0:w463, 5:"温度数据" ("组名称输入（无标题）"), 7:w462, 9:w460) -> ()  [unwired: 2 in, 4 out]
          }
          frame True {
          }
        }
        n257 = Bundle By Name(cluster=w459, "校准时间"=w437) -> (w458:T2)
      }
      frame "Wait" {
        n258 = Unbundle By Name(w469) -> ("校准时间"=w473:timestamp, "温度保存间隔"=w474:dbl)
        n259 = Get Date/Time In Seconds() -> (seconds since 1Jan1904=w477:timestamp)
        n260 = Subtract(x=w474, y=0.015) -> (x-y=w475:dbl)
        n261 = Subtract(x=w477, y=w473) -> (x-y=w464:dbl)
        n262 = Wait (ms)(milliseconds to wait=u32 10 ("等待时间（毫秒）")) -> ()  [unwired: 1 out]
        n263 = Greater Or Equal?(x=w464, y=w475) -> (x >= y?=w476:bool)
        n264 = Select(t=cluster{"消息":string, "消息数据":variant} {"消息"="Save", "消息数据"=variant} ("元素"), s=w476, f=cluster{"消息":string, "消息数据":variant} {"消息"="Wait", "消息数据"=variant} ("元素")) -> (s? t:f=w465:cluster{"消息":string, "消息数据":variant})
        n265 = Enqueue Element(queue=w467, element=w465, error in (no error)=w466) -> ()  [unwired: 1 in, 3 out]
      }
      frame "Stop" {
        n266 = Release Queue(queue=w482, force destroy? (F)=TRUE ("强制销毁？(F)"), error in (no error)=w481) -> ()  [unwired: 3 out]
        n267 = Unbundle By Name(w479) -> ("tdms index"=w478:refnum<k34>)
        n268 = TDMS Close(11:w478) -> ()  [unwired: 1 in, 2 out]
      }
    }
  }
  n269 = Destroy User Event(user event=w22, error in=w20) -> (error out=w23:errorcluster)
  n270 = Unregister For Events(event registration refnum=w21, error in=w23) -> (error out=w14:errorcluster)
  n271 = Merge Errors(w14, w13, w10) -> (w15:errorcluster)
  n272 = call <vilib>:"Simple Error Handler.vi"("error in (no error)"=w15) -> ()  [unwired: 4 in, 5 out]
